vi "CenterOnDisplay.vi"(8 "error in (no error)":errorcluster, 11 "Window in":refnum<class "Window.lvclass">) -> (0 "error out":errorcluster, 3 "Window out":refnum<class "Window.lvclass">)   [LabVIEW 2020, in "GLF.lvlib" / "Window.lvclass"]
uses:
  Window.lvclass
  Window.lvclass/Window.ctl
  <vilib>/Saukko/LV SDL3/Sources/SDL3/Video/Video.lvlib
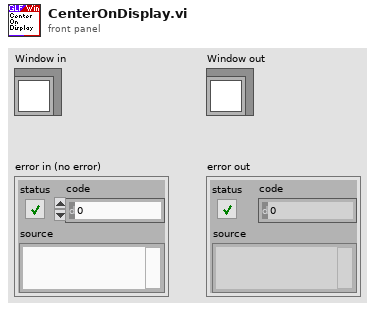
[diagram p1: front panel]
types:
  T1 = typedef "SDL3.lvlib/Video.lvlib/SDL_Window--pointer.ctl" = i64
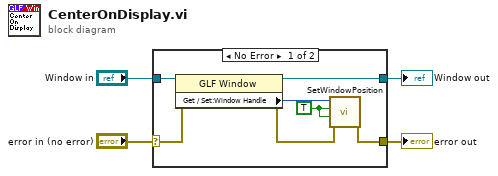
[diagram p0: block diagram]
diagram:
  n1 = case shown="No Error" "error in (no error)" {
    selector: "error in (no error)" -> [w7 w12]
    tunnel: "Window in" -> [w9 w13]
    tunnel: [w10 w12] -> w2
    tunnel: [w8 w13] -> w1
    frame No Error {
      w5 = TRUE ("Center x")
      n2 = property class="GLF Window"(reference=w9, error in=w7) -> (reference out=w8:refnum<class "Window.lvclass">, error out=w11:errorcluster, "Get / Set:Window Handle"=w6:T1)
      n3 = call <vilib>:"SetWindowPosition.vi"("No Error"=w11, "Center y"=w5, "Center x"=w5, "Window [SDL_Window *]"=w6) -> ("Error Out"=w10:errorcluster)  [unwired: 7 in]
    }
    frame Error {
    }
  }
  "Window out" <- w1
  "error out" <- w2
